vi "_incrementTailIndex.vi"(11 "VariantBuffer in":refnum<class "VariantBuffer.lvclass">) -> (3 "VariantBuffer out":refnum<class "VariantBuffer.lvclass">)   [LabVIEW 2013, in "CircularBuffer.lvlib" / "VariantBuffer.lvclass"]
uses:
  VariantBuffer.lvclass
  VariantBuffer.lvclass/VariantBuffer.ctl
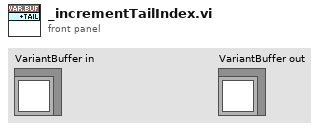
[diagram p1: front panel]
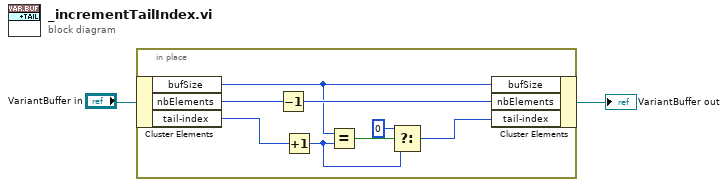
[diagram p0: block diagram]
diagram:
  n1 = in-place {
    n2 = in-place-cluster #1("VariantBuffer in") -> ("bufSize"=w3:i32, "nbElements"=w10:i32, "tail-index"=w4:i32)
    n3 = Decrement(x=w10) -> (x-1=w9:i32)
    n4 = Increment(x=w4) -> (x+1=w7:i32)
    n5 = Equal?(x=w3, y=w7) -> (x = y?=w8:bool)
    n6 = Select(t=0, s=w8, f=w7) -> (s? t:f=w5:i32)
    n7 = in-place-cluster #1("bufSize"=w3, "nbElements"=w9, "tail-index"=w5) -> (→"VariantBuffer out":refnum<class "VariantBuffer.lvclass">)
  }
